vi "UI_Draw_Buttons.vi"(0 "Picture":picture, 1 "Hover":i32=-1, 5 "Specs":T1(array[cluster]), 7 "Values":i32[](array[numeric]), 9 "Dim Groups":bool[](array[boolean]), 11 "error in":errorcluster) -> (4 "New Picture":picture, 15 "error out":errorcluster)   [LabVIEW 2026]
doc: "Specs 배열의 버튼/글자를 둥근 사각형 + 가운데 글자로 그린다.\nValues[Group] = Value면 선택 상태, Hover = 마우스가 올라간 항목 번호, Dim Groups[Group] = 비활성."
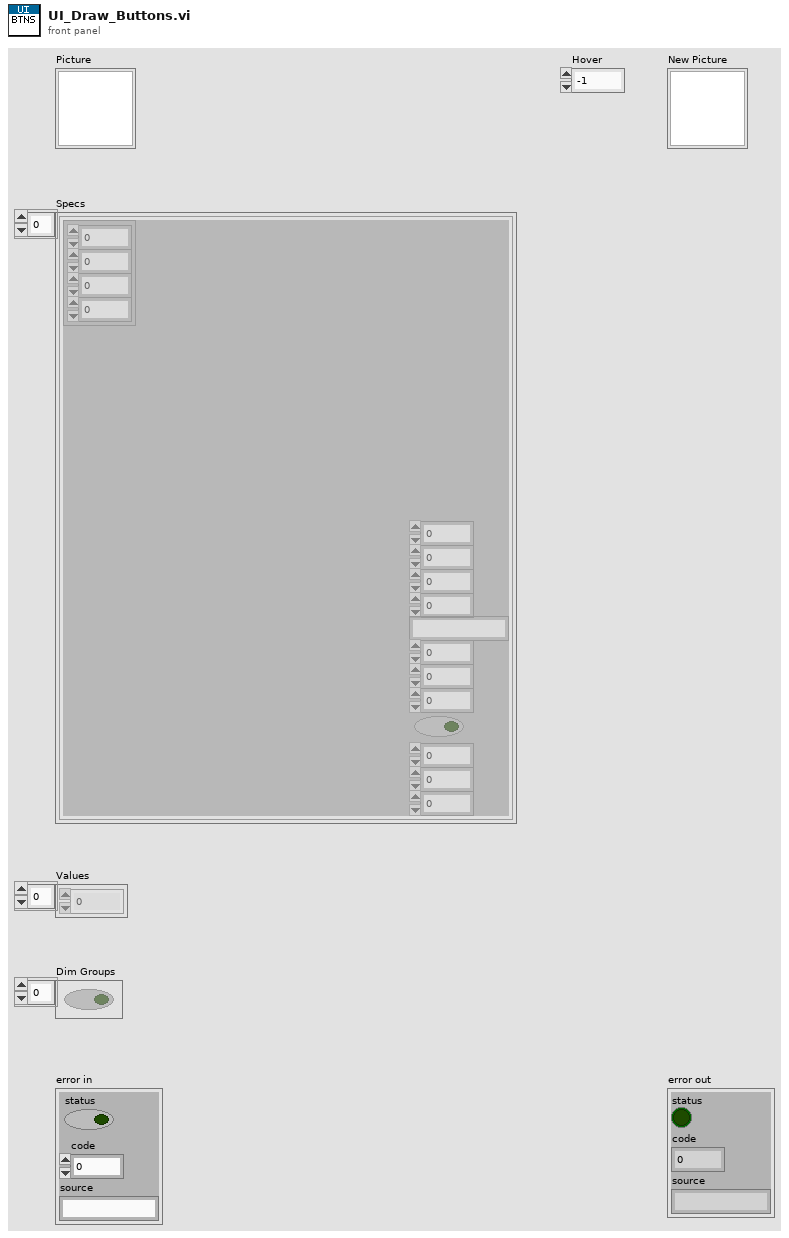
[diagram p1: front panel]
types:
  T1 = cluster{"Rect":cluster{"left":i16, "top":i16, "right":i16, "bottom":i16}, "Fill":u32, "Fill Sel":u32, "Border":u32, "Border Sel":u32, "Text":string, "Text Color":u32, "Text Sel":u32, "Size":i16, "Bold":bool, "Group":i32, "Value":i32, "Radius":i16}[]
  T2 = cluster{"Font Name:":string, "Size":i16, "Strikeout?":bool, "Italic?":bool, "Underline?":bool, "Outline?":bool, "Shadow?":bool, "Bold?":bool}
  T3 = enum16{"User-specified Font", "Application Font", "System Font", "Dialog Font"}
  T4 = cluster{"horizontal":enum16{"left", "center", "right"}, "vertical":enum16{"top", "center", "bottom"}}
  T5 = cluster{"Width":u16, "Style":enum32{"Solid", "Dash", "Dot", "DashDot", "DashDotDot"}}
  T6 = cluster{"left":i16, "top":i16, "right":i16, "bottom":i16}
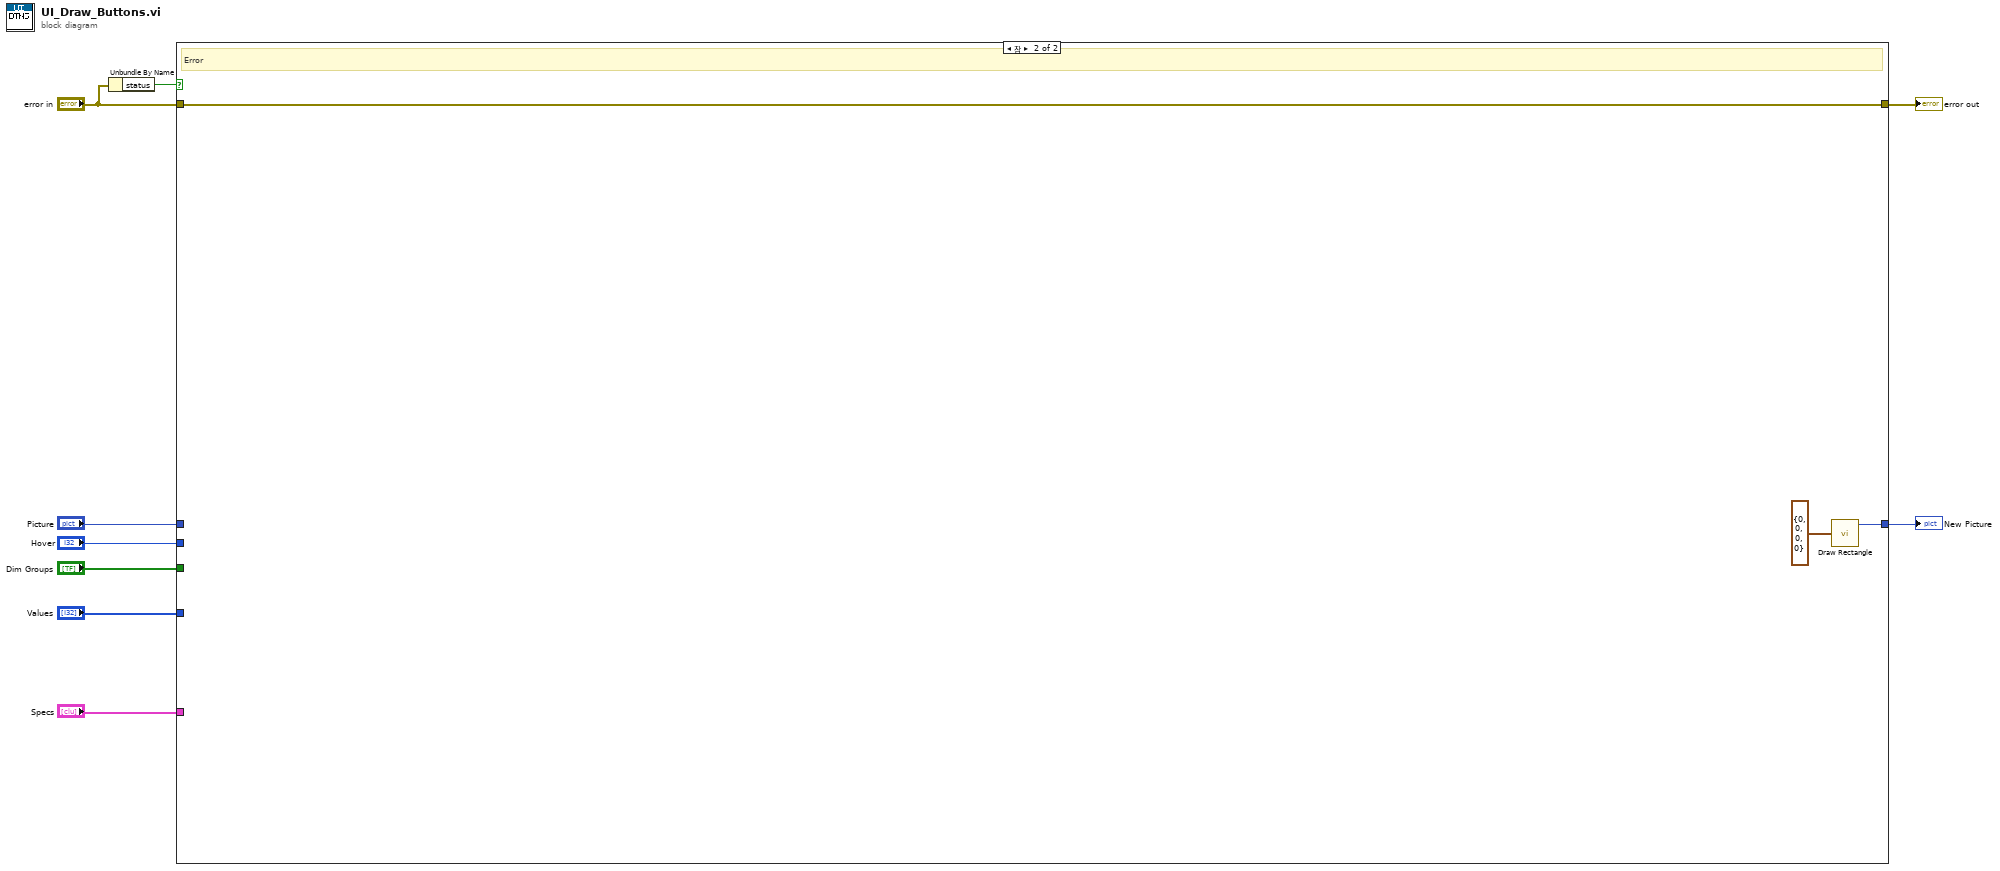
[diagram p0: block diagram]
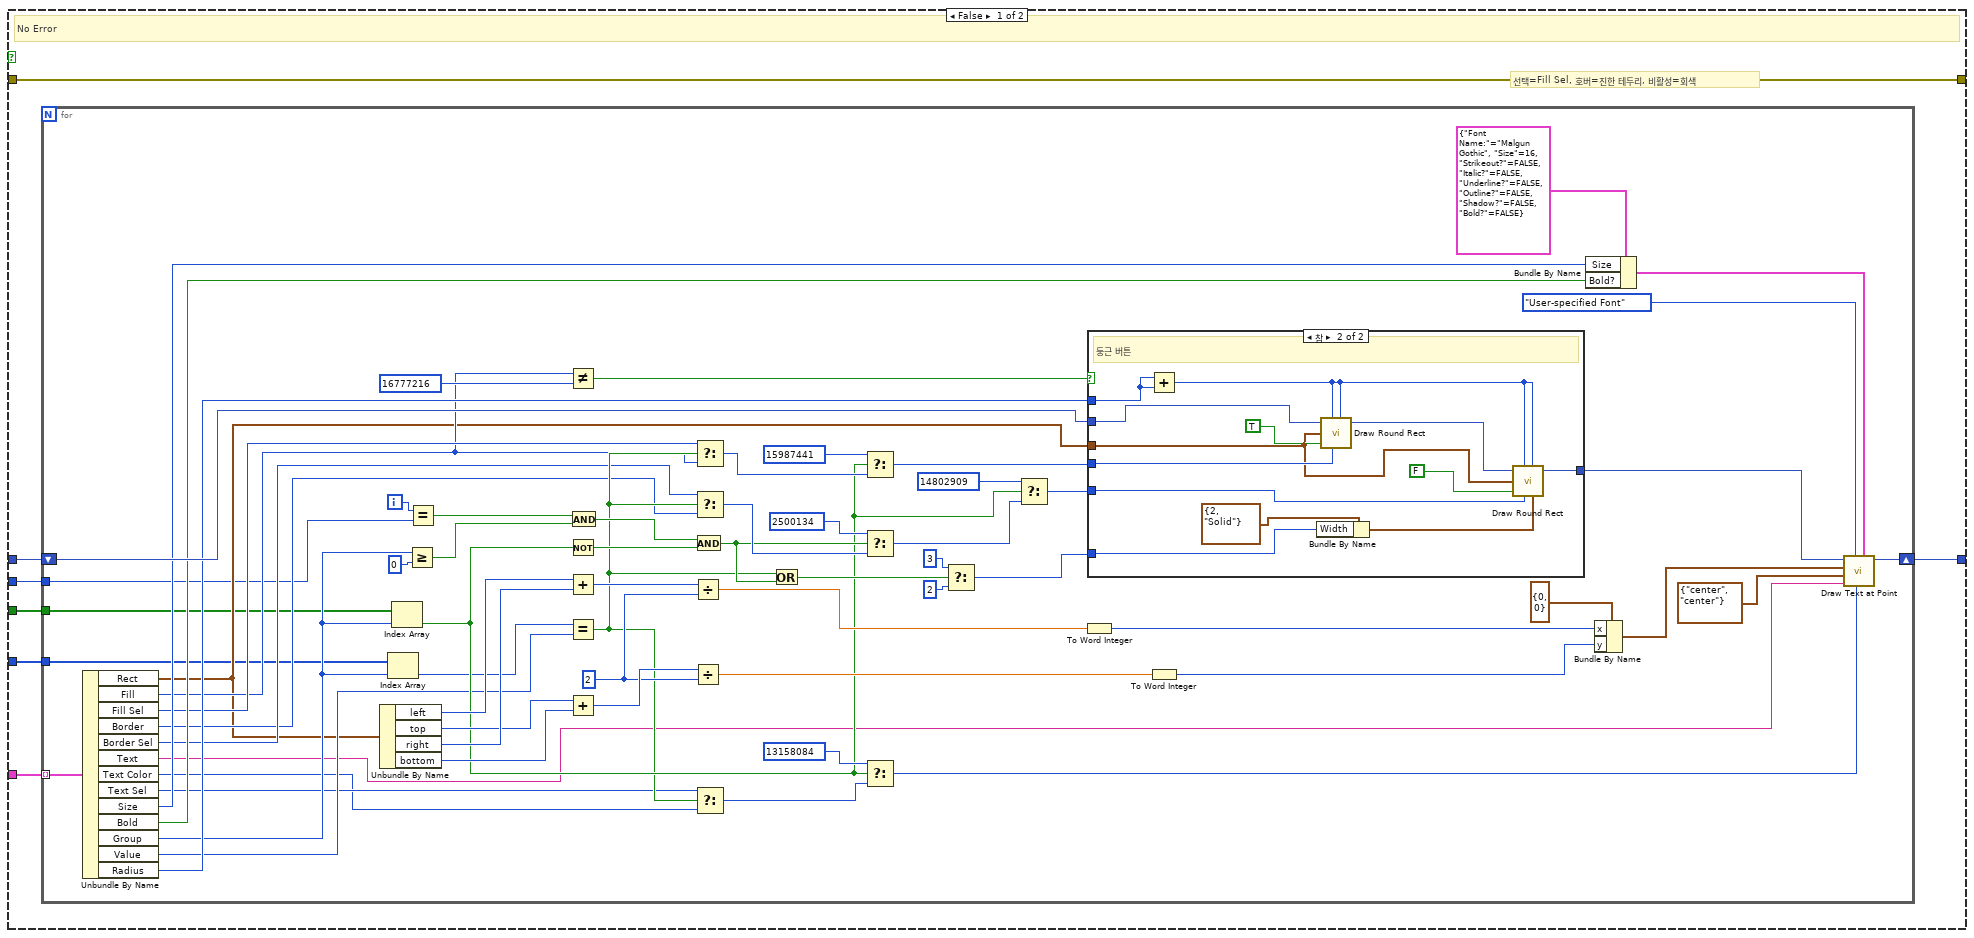
[diagram p2: hidden frame]
diagram:
  n1 = Unbundle By Name("error in") -> ("status"=w7:bool)
  n2 = case shown="참" w7 {
    tunnel: "Picture" -> [w10 _]
    tunnel: "Specs" -> [w11 _]
    tunnel: "Values" -> [w12 _]
    tunnel: "Dim Groups" -> [w13 _]
    tunnel: "Hover" -> [w14 _]
    tunnel: "error in" -> [w15 w95]
    tunnel: [w15 w95] -> w9
    tunnel: [w16 w97] -> w8
    frame False {
      # "선택=Fill Sel, 호버=진한 테두리, 비활성=회색"
      # "No Error"
      n3 = for {
        tunnel: w12 -> [w18]
        tunnel: w13 -> [w19]
        tunnel: w14 -> [w20]
        tunnel: w11 -> [w21] mode=indexing
        shift-right: [w80] -> w16
        shift-left: w10 -> [w61]
        i -> [w17]
        w67 = i16 2
        n4 = Unbundle By Name(w21) -> ("Rect"=w22:T6, "Fill"=w23:u32, "Fill Sel"=w24:u32, "Border"=w25:u32, "Border Sel"=w26:u32, "Text"=w27:string, "Text Color"=w28:u32, "Text Sel"=w29:u32, "Size"=w30:i16, "Bold"=w31:bool, "Group"=w32:i32, "Value"=w33:i32, "Radius"=w34:i16)
        n5 = Unbundle By Name(w22) -> ("left"=w63:i16, "top"=w64:i16, "right"=w65:i16, "bottom"=w66:i16)
        n6 = Index Array(array=w18, index=w32) -> (element=w35:i32)
        n7 = Index Array(array=w19, index=w32) -> (element=w37:bool)
        n8 = Greater Or Equal?(x=w32, y=0) -> (x >= y?=w40:bool)
        n9 = Equal?(x=w17, y=w20) -> (x = y?=w38:bool)
        n10 = Not Equal?(x=w23, y=u32 16777216) -> (x != y?=w60:bool)
        n11 = Not(x=w37) -> (.not. x?=w42:bool)
        n12 = Add(x=w63, y=w65) -> (x+y=w68:i16)
        n13 = Equal?(x=w35, y=w33) -> (x = y?=w36:bool)
        n14 = Add(x=w64, y=w66) -> (x+y=w70:i16)
        n15 = And(x=w38, y=w40) -> (x .and. y?=w41:bool)
        n16 = Divide(x=w68, y=w67) -> (x/y=w69:dbl)
        n17 = Divide(x=w70, y=w67) -> (x/y=w71:dbl)
        n18 = And(x=w41, y=w42) -> (x .and. y?=w43:bool)
        n19 = Select(t=w24, s=w36, f=w23) -> (s? t:f=w45:u32)
        n20 = Select(t=w26, s=w36, f=w25) -> (s? t:f=w49:u32)
        n21 = Select(t=w29, s=w36, f=w28) -> (s? t:f=w53:u32)
        n22 = Or(x=w36, y=w43) -> (x .or. y?=w55:bool)
        n23 = Select(t=u32 15987441, s=w37, f=w45) -> (s? t:f=w46:u32)
        n24 = Select(t=u32 2500134, s=w43, f=w49) -> (s? t:f=w50:u32)
        n25 = Select(t=u32 13158084, s=w37, f=w53) -> (s? t:f=w54:u32)
        n26 = Select(t=u16 3, s=w55, f=u16 2) -> (s? t:f=w58:u16)
        n27 = Select(t=u32 14802909, s=w37, f=w50) -> (s? t:f=w51:u32)
        n28 = To Word Integer(number=w69) -> (16bit integer=w72:i16)
        n29 = case shown="참" w60 {
          tunnel: w61 -> [w81 w82]
          tunnel: w22 -> [_ w83]
          tunnel: w34 -> [_ w86]
          tunnel: w46 -> [_ w84]
          tunnel: w51 -> [_ w85]
          tunnel: w58 -> [_ w87]
          tunnel: [w81 w94] -> w62
          frame False {
            # "글자만"
          }
          frame True {
            # "둥근 버튼"
            n30 = Add(x=w86, y=w86) -> (x+y=w88:i16)
            n31 = Bundle By Name(cluster=T5 {"Width"=2, "Style"=enum."Solid"}, "Width"=w87) -> (w93:T5)
            n32 = call <vilib>:"Draw Round Rect.vi"("picture"=w82, "oval width"=w88, "rect"=w83, "fill?(F)"=TRUE, "color(black)"=w84, "oval height"=w88) -> ("new picture"=w90:picture)  [unwired: 3 in]
            n33 = call <vilib>:"Draw Round Rect.vi"("picture"=w90, "oval width"=w88, "rect"=w83, "fill?(F)"=FALSE, "color(black)"=w85, "oval height"=w88, "pen"=w93) -> ("new picture"=w94:picture)  [unwired: 2 in]
          }
        }
        n34 = To Word Integer(number=w71) -> (16bit integer=w73:i16)
        n35 = Bundle By Name(cluster=T2 {"Font Name:"="Malgun Gothic", "Size"=16, "Strikeout?"=FALSE, "Italic?"=FALSE, "Underline?"=FALSE, "Outline?"=FALSE, "Shadow?"=FALSE, "Bold?"=FALSE}, "Size"=w30, "Bold?"=w31) -> (w79:T2)
        n36 = Bundle By Name(cluster=cluster{"x":i16, "y":i16} {"x"=0, "y"=0}, "x"=w72, "y"=w73) -> (w75:cluster{"x":i16, "y":i16})
        n37 = call <vilib>:"Draw Text at Point.vi"("[user-specified font]"=w79, "text color(black)"=w54, "desired font(Application)"=T3."User-specified Font", "text"=w27, "alignment(left, top)"=T4 {"horizontal"=enum."center", "vertical"=enum."center"}, "origin"=w75, "picture"=w62) -> ("new picture"=w80:picture)  [unwired: 3 in, 1 out]
      }
    }
    frame True {
      # "Error"
      n38 = call <vilib>:"Draw Rectangle.vi"("rect"=T6 {"left"=0, "top"=0, "right"=0, "bottom"=0}) -> ("new picture"=w97:picture)  [unwired: 8 in]
    }
  }
  "New Picture" <- w8
  "error out" <- w9
